vi "mupRelease.vi"(8 "error in (no error)":errorcluster, 11 "hParser in":u64) -> (0 "error out":errorcluster)   [LabVIEW 2018, in "mupLib.lvlib"]
doc: "Close the muParser instance."
uses:
  mupLib.lvlib
  libmuparser-lv.dll
panel:
  # "Close the muParser instance."
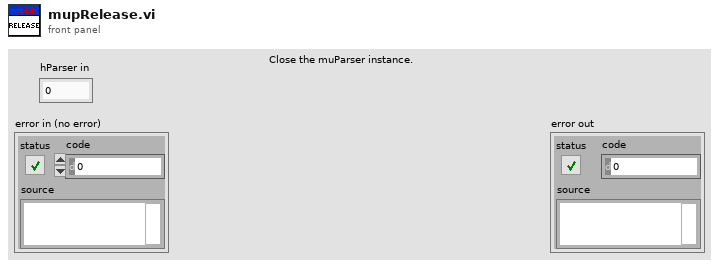
[diagram p1: front panel]
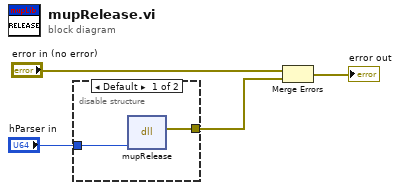
[diagram p0: block diagram]
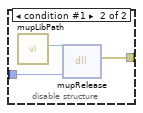
[diagram p2: hidden frame]
diagram:
  n1 = disable-structure shown="Default" {
    disable-tunnel: [w6 w9] -> w3
    disable-tunnel: "hParser in" -> [w5 w8]
    frame condition #0 (active) {
      n2 = dll-call lib="C:/Users/leonidas/Documents/GitHub/LV-muParser/mupLib/libmuparser-lv.dll" fn="mupRelease"("hParser"=w5) -> (error out=w6:errorcluster)  [unwired: 5 in, 1 out]
    }
    frame condition #1 {
      n3 = call "mupLibPath.vi"() -> ("libmuparser path"=w7:path)  [unwired: 11 in]
      n4 = dll-call lib="C:/Users/leonidas/Documents/GitHub/LV-muParser/mupLib/libmuparser-lv.dll" fn="mupRelease"(path in=w7, "hParser"=w8) -> (error out=w9:errorcluster)  [unwired: 4 in, 1 out]
    }
  }
  n5 = Merge Errors("error in (no error)", w3) -> (→"error out":errorcluster)
